vi "Add Node.vi"(8 "error in (no error)":errorcluster, 9 "Assertions":T1[](array[typedef]), 10 "Test Node":T2, 11 "Test Result in":refnum<class "Test Result.lvclass">) -> (0 "error out":errorcluster, 3 "Test Result out":refnum<class "Test Result.lvclass">)   [LabVIEW 2020, in "Caraya.lvlib" / "Test Result.lvclass"]
uses:
  Test Result.lvclass
  Test Node.ctl
  Test Registration Data.ctl
  Assert Event Data.ctl
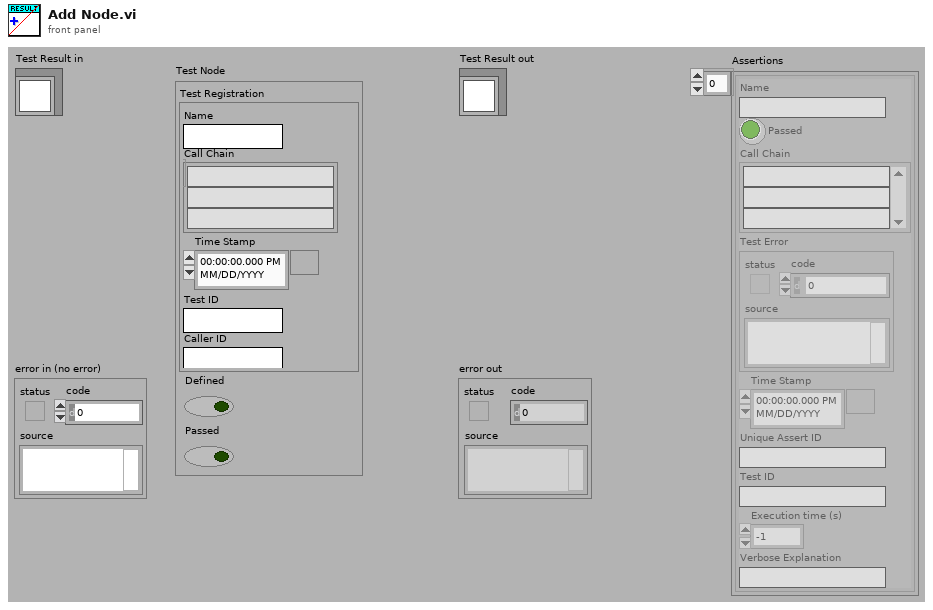
[diagram p1: front panel]
types:
  T1 = typedef "Caraya.lvlib/Test Result.lvclass/Assert Event Data.ctl" = cluster{"Name":string, "Passed":bool, "Call Chain":string[], "Test Error":errorcluster, "Time Stamp":timestamp, "Unique Assert ID":string, "Test ID":string, "Execution time (s)":dbl, "Verbose Explanation":string}
  T2 = typedef "Caraya.lvlib/Test Result.lvclass/Test Node.ctl" = cluster{"Test Registration":T3, "Defined":bool, "Passed":bool}
  T3 = typedef "Caraya.lvlib/Test Result.lvclass/Test Registration Data.ctl" = cluster{"Name":string, "Call Chain":string[], "Time Stamp":timestamp, "Test ID":string, "Caller ID":string}
  T4 = typedef "Caraya.lvlib/Test Result.lvclass/Assert Event Data (Extended).ctl" = cluster{"name":string, "passed":bool, "call-chain":string[], "test-error":errorcluster, "timestamp":timestamp, "assert-id":string, "test-id":string, "time":dbl, "message":string, "properties":variant, "measurements":variant, "user-defined":variant}
  T5 = typedef "Caraya.lvlib/Test Result.lvclass/Test Node (Extended).ctl" = cluster{"Test Registration":T3, "Defined":bool, "Passed":bool, "properties":variant}
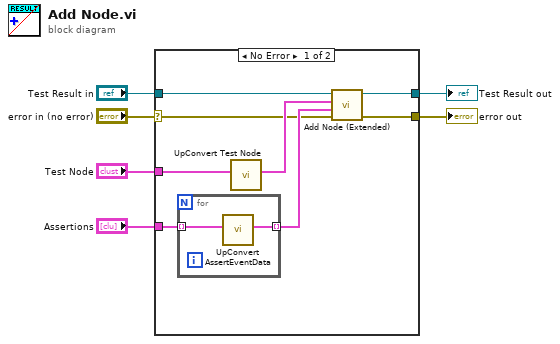
[diagram p0: block diagram]
diagram:
  n1 = case shown="No Error" "error in (no error)" {
    selector: "error in (no error)" -> [w8 w18]
    tunnel: [w7 w18] -> w5
    tunnel: [w9 w17] -> w3
    tunnel: "Test Result in" -> [w10 w17]
    tunnel: "Test Node" -> [w13 _]
    tunnel: "Assertions" -> [w14 _]
    frame No Error {
      n2 = for {
        tunnel: [w15] -> w12 mode=indexing
        tunnel: w14 -> [w16] mode=indexing
        n3 = call "UpConvert AssertEventData.vi"("Assert Event Data"=w16) -> ("Assert Event Data (Extended)"=w15:T4)  [unwired: 10 in]
      }
      n4 = call "UpConvert Test Node.vi"("Test Node"=w13) -> ("Test Node (Extended)"=w11:T5)  [unwired: 10 in]
      n5 = call "Add Node (Extended).vi"("error in (no error)"=w8, "Assertions"=w12, "Test Node"=w11, "Test Result in"=w10) -> ("error out"=w7:errorcluster, "Test Result out"=w9:refnum<class "Test Result.lvclass">)  [unwired: 6 in]
    }
    frame Error {
    }
  }
  "error out" <- w5
  "Test Result out" <- w3
